vi "Measurement Logic.vi"(8 "error in":errorcluster, 9 "measurement configuration":T2={"DPE Project File Path"="", "Site"=1, "DUT Bring Up"="", "Apply TDR?"=FALSE, "List-Patterns"=[], "List-Current Measurement Pins"=[]}, 10 "measure call context in":refnum<class "Measure Call Context.lvclass">) -> (0 "error out":errorcluster, 1 "measurement results":T1={"All Pass?"=FALSE, "Results"="Empty"}, 2 "measure call context out":refnum<class "Measure Call Context.lvclass">)   [LabVIEW 2025, in "Digital Pattern Sequencer.lvclass"]
doc: "Contains the core logic for executing the measurement."
uses:
  Digital Pattern Sequencer.lvclass
  Digital Pattern Sequencer.lvclass/Digital Pattern Sequencer.ctl
  Measurement Results.ctl
  <vilib>/Plug-In SDKs/Measurements/Measure Call Context/Measure Call Context.lvclass
  Measurement Configuration.ctl
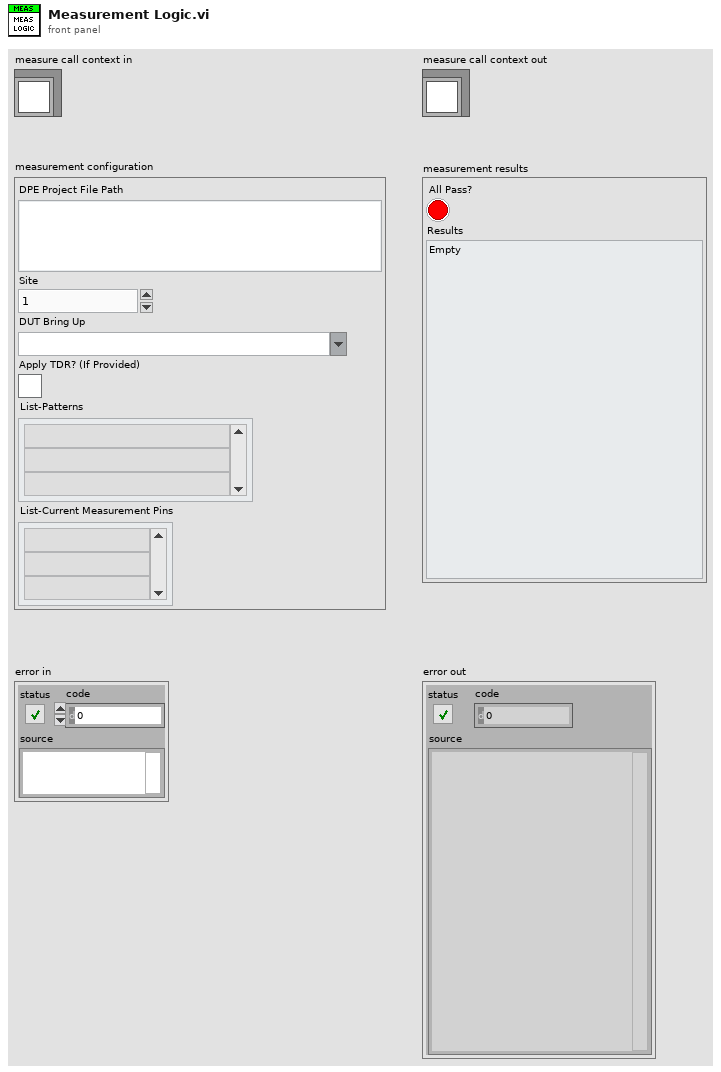
[diagram p1: front panel]
types:
  T1 = typedef "Digital Pattern Sequencer.lvclass/Measurement Results.ctl" = cluster{"All Pass?":bool, "Results":string}
  T2 = typedef "Digital Pattern Sequencer.lvclass/Measurement Configuration.ctl" = cluster{"DPE Project File Path":string, "Site":i32, "DUT Bring Up":string, "Apply TDR?":bool, "List-Patterns":string[], "List-Current Measurement Pins":string[]}
  T3 = typedef "Event Messenger-bool.lvlib/))Channel.ctl" = refnum<queue>
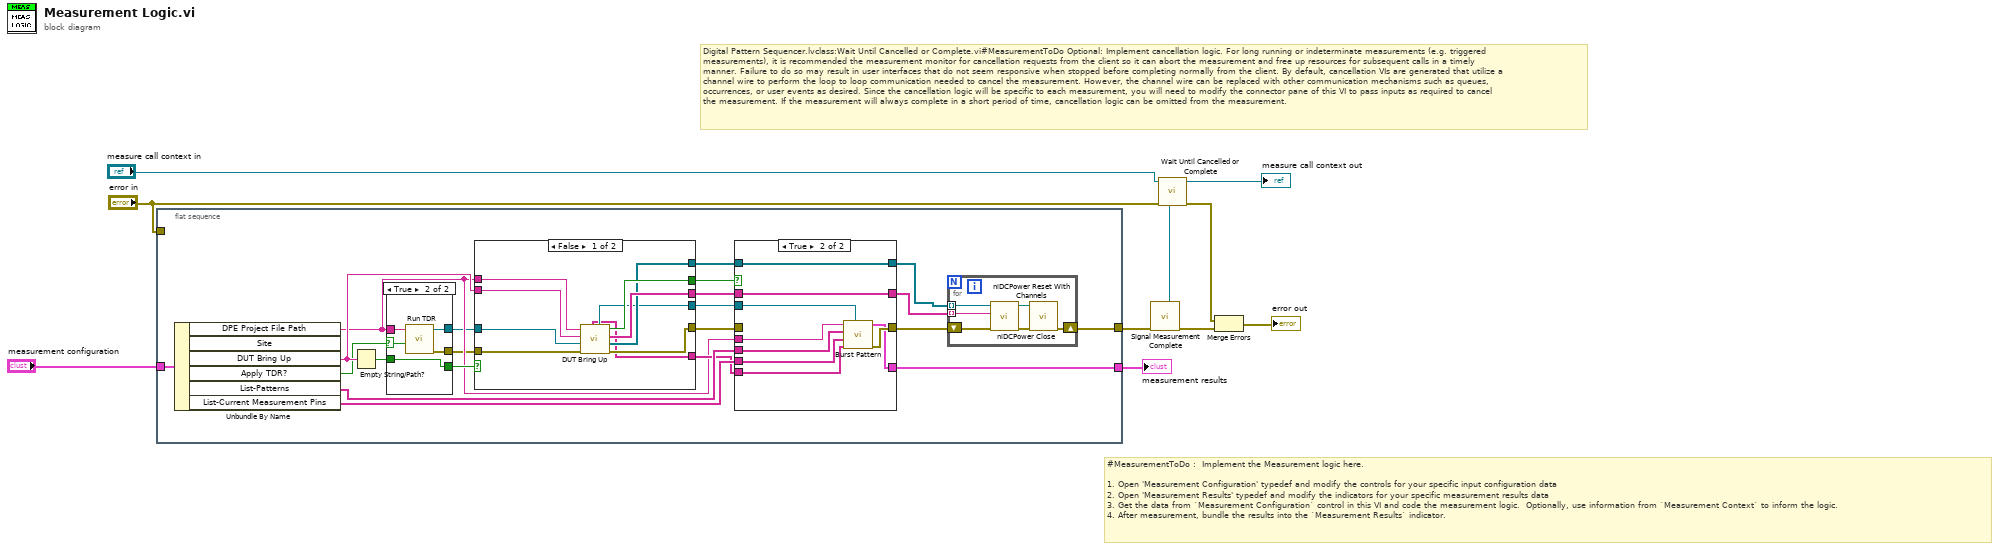
[diagram p0: block diagram]
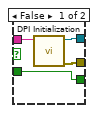
[diagram p2: hidden frame]
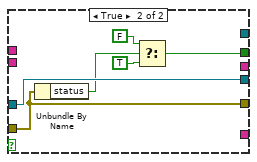
[diagram p3: hidden frame]
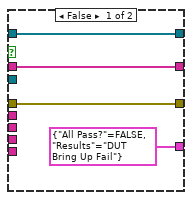
[diagram p4: hidden frame]
diagram:
  # "Digital Pattern Sequencer.lvclass:Wait Until Cancelled or Complete.vi#MeasurementToDo Optional: Implement cancellation logic. For long running or indeterminate measurements (e.g. triggered measurements), it is recommended the measurement monitor for cancellation requests from the client so it can abort the measurement and free up resources for subsequent calls in a timely manner. Failure to do so may result in user interfaces that do not seem responsive when stopped before completing normally from the client. By default, cancellation VIs are generated that utilize a channel wire to perform the loop to loop communication needed to cancel the measurement. However, the channel wire can be replaced with other communication mechanisms such as queues, occurrences, or user events as desired. Since the cancellation logic will be specific to each measurement, you will need to modify the connector pane of this VI to pass inputs as required to cancel the measurement. If the measurement will always complete in a short period of time, cancellation logic can be omitted from the measurement."
  # "#MeasurementToDo :  Implement the Measurement logic here.\n\n1. Open 'Measurement Configuration' typedef and modify the controls for your specific input configuration data\n2. Open 'Measurement Results' typedef and modify the indicators for your specific measurement results data\n3. Get the data from `Measurement Configuration` control in this VI and code the measurement logic.  Optionally, use information from `Measurement Context` to inform the logic.\n4. After measurement, bundle the results into the `Measurement Results` indicator."
  n1 = flat-sequence {
    tunnel: "measurement configuration" -> [w31]
    tunnel: [w28] -> w9
    tunnel: "error in" -> [_]
    tunnel: [w19] -> w5
    frame #0 {
      n2 = Unbundle By Name(w31) -> ("DPE Project File Path"=w13:string, "DUT Bring Up"=w25:string, "Apply TDR?"=w15:bool, "List-Patterns"=w29:string[], "List-Current Measurement Pins"=w30:string[])  [unwired: 1 out]
      n3 = Empty String/Path?(string/path=w25) -> (empty?=w16:bool)
      n4 = case shown="True" w15 {
        selector: w15 -> [_ w45]
        tunnel: w16 -> [w41 w46]
        tunnel: [w41 w46] -> w14
        tunnel: w13 -> [w40 w44]
        tunnel: [w39 w43] -> w12
        tunnel: [w38 w42] -> w11
        frame False {
          n5 = call "DPI Initialization.vi"("DPE Project File Path"=w40) -> ("error out"=w38:errorcluster, "DPI Instrument Name"=w39:refnum<k15>)  [unwired: 9 in]
        }
        frame True {
          n6 = call "Run TDR.vi"("Apply TDR?"=w45, "DPE Project File Path"=w44) -> ("error out"=w42:errorcluster, "DPI Instrument Name"=w43:refnum<k15>)  [unwired: 8 in]
        }
      }
      n7 = case shown="False" w14 {
        tunnel: w13 -> [w56 _]
        tunnel: [w55 w61] -> w27
        tunnel: [w54 w57] -> w26
        tunnel: w25 -> [w53 _]
        tunnel: [w52 _] -> w24
        tunnel: [w51 _] -> w23
        tunnel: [w50 w62] -> w18
        tunnel: [w49 _] -> w17
        tunnel: w12 -> [w48 w62]
        tunnel: w11 -> [w47 w61]
        frame False {
          n8 = call "DUT Bring Up.vi"("error in"=w47, "DPI Instrument Name"=w48, "DUT Bring Up"=w53, "DPE Project File Path"=w56) -> ("error out"=w55:errorcluster, "DUT Bring Up Vcc Resource"=w51:refnum<k15>[], "DUT Bring Up DCPower Channels"=w52:string[], "DUT Bring Up PASS?"=w54:bool, "DPI Instrument Name"=w50:refnum<k15>, "DUT Bring Up Pin"=w49:string[])  [unwired: 2 in]
        }
        frame True {
          n9 = Unbundle By Name(w61) -> ("status"=w60:bool)
          n10 = Select(t=FALSE ("DUT Bring Up PASS?"), s=w60, f=TRUE ("DUT Bring Up PASS?")) -> (s? t:f=w57:bool)
        }
      }
      n11 = case shown="True" w26 {
        tunnel: [w65 w75] -> w20
        tunnel: w30 -> [_ w74]
        tunnel: w29 -> [_ w73]
        tunnel: [T1 {"All Pass?"=FALSE, "Results"="DUT Bring Up Fail"} ("Measurement Results") w72] -> w28
        tunnel: w13 -> [_ w71]
        tunnel: w27 -> [w65 _]
        tunnel: w24 -> [w63 w70]
        tunnel: w23 -> [w64 w69]
        tunnel: [w63 w70] -> w22
        tunnel: [w64 w69] -> w21
        tunnel: w18 -> [_ w68]
        tunnel: w17 -> [_ w67]
        frame False {
        }
        frame True {
          n12 = call "Burst Pattern.vi"("DPI Instrument Name"=w68, "DUT Bring Up Pins"=w67, "List-Current Measurement Pins"=w74, "List-Patterns"=w73, "DPE Project File Path"=w71) -> ("error out"=w75:errorcluster, "Measurement Results"=w72:T1)  [unwired: 5 in]
        }
      }
      n13 = for {
        tunnel: w22 -> [w35] mode=indexing
        tunnel: w21 -> [w34] mode=indexing
        shift-right: [w32] -> w19
        shift-left: w20 -> [w33]
        n14 = call <instrlib>:"niDCPower Reset With Channels.vi"("error in (no error)"=w33, "channel name"=w35, "instrument handle"=w34) -> ("error out"=w37:errorcluster, "instrument handle out"=w36:refnum<k15>)  [unwired: 7 in]
        n15 = call <instrlib>:"niDCPower Close.vi"("error in (no error)"=w37, "instrument handle"=w36) -> ("error out"=w32:errorcluster)  [unwired: 9 out]
      }
    }
  }
  n16 = call "Signal Measurement Complete.vi"("error in (no error)"=w5) -> ("error out"=w3:errorcluster, "done channel"=w4:T3)  [unwired: 9 in]
  n17 = call "Wait Until Cancelled or Complete.vi"("done channel"=w4, "error in (no error)"="error in", "measure call context in"="measure call context in") -> ("error out"=w2:errorcluster, "measure call context out"=→"measure call context out":refnum<class "Measure Call Context.lvclass">)  [unwired: 7 in]
  n18 = Merge Errors(w2, w3) -> (→"error out":errorcluster)
  "measurement results" <- w9
